vi "Test - String Arrays Equal.vi"(8 "error in":errorcluster, 10 "Expected":string[](array[string]), 11 "Actual":string[](array[string])) -> (0 "error out":errorcluster, 3 "Equal?":bool)   [LabVIEW 2026]
doc: "Test helper. Equal? is TRUE when Actual and Expected have the same number of elements and every element is equal (case sensitive, in order). error in is passed through unchanged.\n\nGenerated by: Claude"
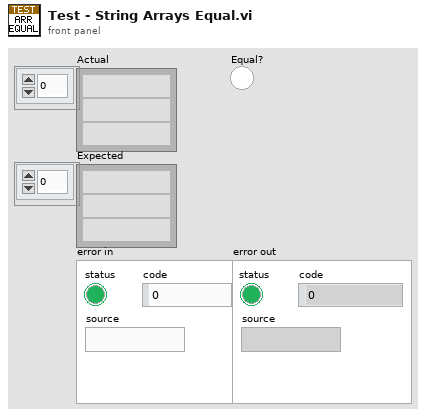
[diagram p1: front panel]
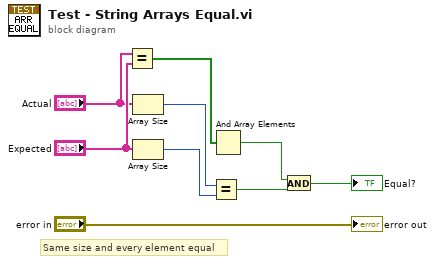
[diagram p0: block diagram]
diagram:
  # "Same size and every element equal"
  n1 = Equal?(x="Actual", y="Expected") -> (x = y?=w5:bool[])
  n2 = Array Size(array="Actual") -> (size(s)=w7:i32)
  n3 = Array Size(array="Expected") -> (size(s)=w8:i32)
  n4 = Equal?(x=w7, y=w8) -> (x = y?=w9:bool)
  n5 = And Array Elements(Boolean array=w5) -> (logical AND=w6:bool)
  n6 = And(x=w6, y=w9) -> (x .and. y?=→"Equal?":bool)
  "error out" <- "error in"
